vi "SeqEditor_PanelResize.vi"(8 "error in (no error)":errorcluster, 11 "NLTest in":refnum<class "NLTest.lvclass">) -> (0 "error out":errorcluster, 3 "NLTest out":refnum<class "NLTest.lvclass">)   [LabVIEW 2017, in "NLTest.lvclass"]
uses:
  NLTest.lvclass
  NLTest.lvclass/NLTest.ctl
  <vilib>/Utility/miscctls.llb/LVRowAndColumnTypeDef.ctl
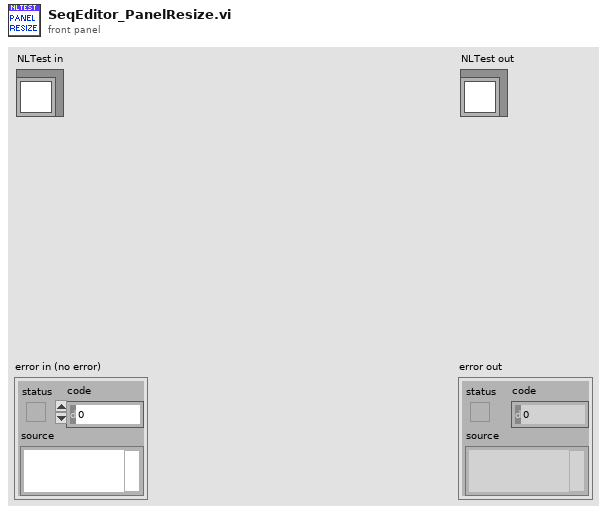
[diagram p1: front panel]
types:
  T1 = typedef "LVRowAndColumnTypeDef.ctl" = cluster{"Row":i32, "Column":i32}
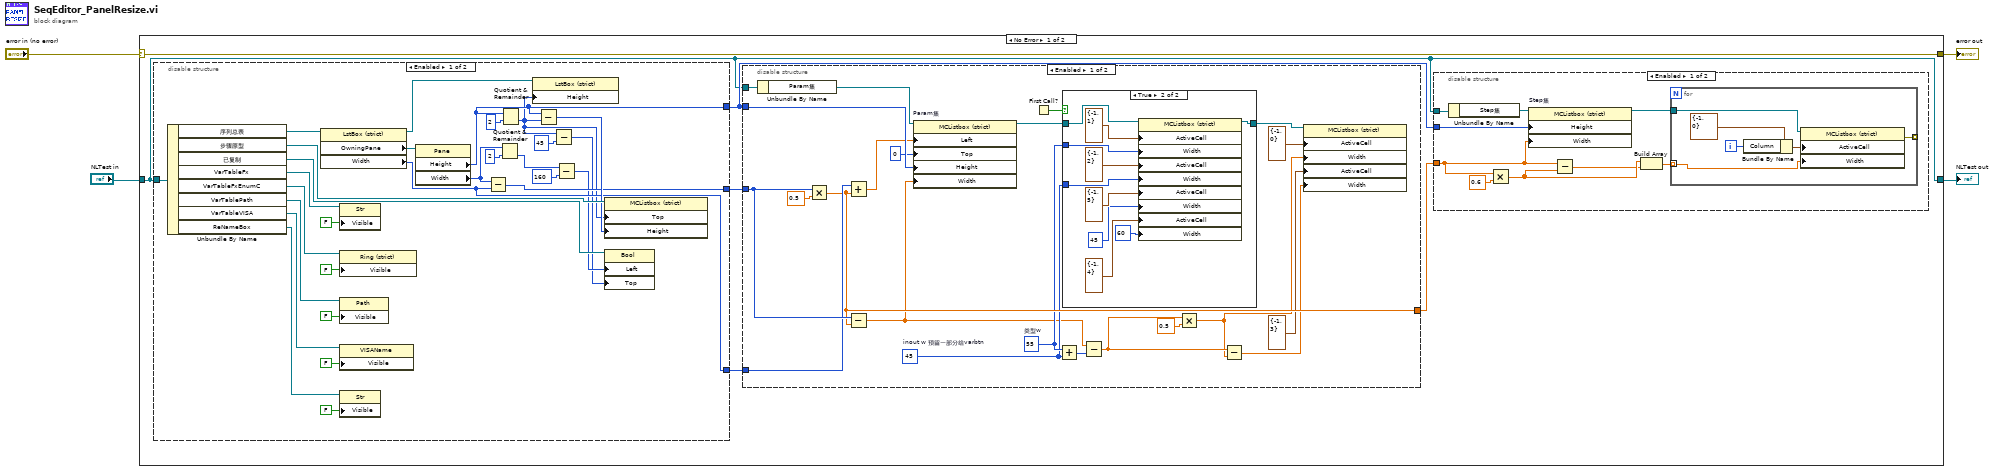
[diagram p0: block diagram]
diagram:
  n1 = case shown="No Error" "error in (no error)" {
    selector: "error in (no error)" -> [w10 w89]
    tunnel: [w10 w89] -> w3
    tunnel: [w5 w88] -> w1
    tunnel: "NLTest in" -> [w5 w88]
    frame No Error {
      n2 = disable-structure shown="Enabled" {
        disable-tunnel: w5 -> [w66 _]
        disable-tunnel: [w65 _] -> w9
        disable-tunnel: [w64 _] -> w8
        disable-tunnel: [w63 _] -> w7
        frame Enabled {
          n3 = Unbundle By Name(w66) -> ("序列总表"=w72:refnum<vi>, "步骤原型"=w68:refnum<vi>, "已复制"=w62:refnum<vi>, "VarTableFx"=w53:refnum<vi>, "VarTableFxEnumC"=w50:refnum<vi>, "VarTablePath"=w48:refnum<vi>, "VarTableVISA"=w46:refnum<vi>, "ReNameBox"=w44:refnum<vi>)
          n4 = property class="LstBox (strict)"(reference=w72) -> (reference out=w69:refnum<vi>, "OwningPane"=w71:refnum<vi>, "Width"=w63:u32)  [unwired: 1 in, 1 out]
          n5 = property class="Str"(reference=w53, "Visible"=FALSE) -> ()  [unwired: 1 in, 2 out]
          n6 = property class="Ring (strict)"(reference=w50, "Visible"=FALSE) -> ()  [unwired: 1 in, 2 out]
          n7 = property class="Path"(reference=w48, "Visible"=FALSE) -> ()  [unwired: 1 in, 2 out]
          n8 = property class="VISAName"(reference=w46, "Visible"=FALSE) -> ()  [unwired: 1 in, 2 out]
          n9 = property class="Str"(reference=w44, "Visible"=FALSE) -> ()  [unwired: 1 in, 2 out]
          n10 = property class="Pane"(reference=w71) -> ("Height"=w65:u32, "Width"=w60:u32)  [unwired: 1 in, 2 out]
          n11 = Subtract(x=w60, y=w63) -> (x-y=w64:u32)
          n12 = Quotient & Remainder(x=w60, y=u32 2) -> (floor(x/y)=w59:u32)  [unwired: 1 out]
          n13 = Quotient & Remainder(x=w65, y=u32 2) -> (floor(x/y)=w58:u32)  [unwired: 1 out]
          n14 = property class="LstBox (strict)"(reference=w69, "Height"=w58) -> ()  [unwired: 1 in, 2 out]
          n15 = Subtract(x=w65, y=w58) -> (x-y=w67:u32)
          n16 = Subtract(x=w58, y=u32 45) -> (x-y=w55:u32)
          n17 = Subtract(x=w59, y=u32 160) -> (x-y=w57:u32)
          n18 = property class="MCListbox (strict)"(reference=w68, "Top"=w58, "Height"=w67) -> ()  [unwired: 1 in, 2 out]
          n19 = property class="Bool"(reference=w62, "Left"=w57, "Top"=w55) -> ()  [unwired: 1 in, 2 out]
        }
        frame Disabled {
        }
      }
      n20 = disable-structure shown="Enabled" {
        disable-tunnel: w5 -> [w32 _]
        disable-tunnel: w9 -> [w29 _]
        disable-tunnel: w8 -> [w28 _]
        disable-tunnel: w7 -> [w26 _]
        disable-tunnel: [w24 _] -> w6
        frame Enabled {
          w19 = u32 45  # inout w 预留一部分给varbtn
          w20 = u32 55  # 类型w
          n21 = Unbundle By Name(w32) -> ("Param集"=w31:refnum<vi>)
          n22 = Multiply(x=w28, y=0.5) -> (x*y=w24:dbl)
          n23 = Add(x=w26, y=w24) -> (x+y=w27:dbl)
          n24 = Subtract(x=w28, y=w24) -> (x-y=w17:dbl)
          n25 = property on="Param集" class="MCListbox (strict)"(reference=w31, "Left"=w27, "Top"=0 ("Position:Top"), "Height"=w29, "Width"=w17) -> (reference out=w23:refnum<vi>)  [unwired: 1 in, 1 out]
          n26 = First Call?() -> (First Call?: T/F=w22:bool)
          n27 = Add(x=w20, y=w19) -> (x+y=w18:u32)
          n28 = case shown="True" w22 {
            tunnel: w23 -> [w33 w43]
            tunnel: [w33 w38] -> w21
            tunnel: w20 -> [_ w35]
            tunnel: w19 -> [_ w34]
            frame False {
            }
            frame True {
              n29 = property class="MCListbox (strict)"(reference=w43, "ActiveCell"=T1 {"Row"=-1, "Column"=1} ("Active Cell:Active Cell"), "Width"=w35, "ActiveCell"=T1 {"Row"=-1, "Column"=2} ("Active Cell:Active Cell"), "Width"=w34, "ActiveCell"=T1 {"Row"=-1, "Column"=5} ("Active Cell:Active Cell"), "Width"=u32 45 ("Active Cell:Cell Size:Width"), "ActiveCell"=T1 {"Row"=-1, "Column"=4} ("Active Cell:Active Cell"), "Width"=u32 60 ("Active Cell:Cell Size:Width")) -> (reference out=w38:refnum<vi>)  [unwired: 1 in, 1 out]
            }
          }
          n30 = Subtract(x=w17, y=w18) -> (x-y=w15:dbl)
          n31 = Multiply(x=w15, y=0.5) -> (x*y=w12:dbl)
          n32 = Subtract(x=w15, y=w12) -> (x-y=w11:dbl)
          n33 = property class="MCListbox (strict)"(reference=w21, "ActiveCell"=T1 {"Row"=-1, "Column"=0} ("Active Cell:Active Cell"), "Width"=w12, "ActiveCell"=T1 {"Row"=-1, "Column"=3} ("Active Cell:Active Cell"), "Width"=w11) -> ()  [unwired: 1 in, 2 out]
        }
        frame Disabled {
        }
      }
      n34 = disable-structure shown="Enabled" {
        disable-tunnel: w9 -> [w81 _]
        disable-tunnel: w6 -> [w77 _]
        disable-tunnel: w5 -> [w74 _]
        frame Enabled {
          n35 = Unbundle By Name(w74) -> ("Step集"=w73:refnum<vi>)
          n36 = Multiply(x=w77, y=0.6) -> (x*y=w76:dbl)
          n37 = property on="Step集" class="MCListbox (strict)"(reference=w73, "Height"=w81, "Width"=w77) -> (reference out=w80:refnum<vi>)  [unwired: 1 in, 1 out]
          n38 = Subtract(x=w77, y=w76) -> (x-y=w75:dbl)
          n39 = Build Array(w76, w75) -> (w78:dbl[])
          n40 = for {
            tunnel: [w85] -> _ mode=indexing
            tunnel: w80 -> [w83]
            tunnel: w78 -> [w82] mode=indexing
            i -> [w86]
            n41 = Bundle By Name(cluster=T1 {"Row"=-1, "Column"=0} ("编辑位置"), "Column"=w86) -> (w87:T1)
            n42 = property class="MCListbox (strict)"(reference=w83, "ActiveCell"=w87, "Width"=w82) -> (error out=w85:errorcluster)  [unwired: 1 in, 1 out]
          }
        }
        frame Disabled {
        }
      }
    }
    frame Error {
    }
  }
  "error out" <- w3
  "NLTest out" <- w1
